vi "UDP Date Time and Match Status to RPI.vi"(6 "Address":u32, 9 "Port":u16, 10 "port":refnum<k16>) -> ()   [LabVIEW 2025]
uses:
  <vilib>/Rock Robotics/SystemInterfaces/NetworkCommunication/NetComm_MatchType.ctl
  <vilib>/Rock Robotics/WPI/DriverStation/WPI_DriverStationRobotMode2.ctl
panel:
  out "Match Type":T1
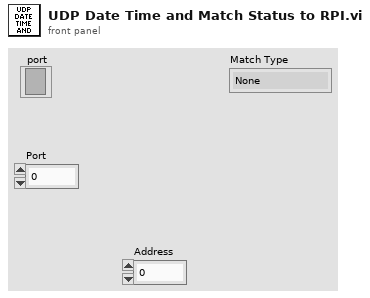
[diagram p1: front panel]
types:
  T1 = typedef "NetComm_MatchType.ctl" = enum32{"None", "Practice", "Qualification", "Elimination"}
  T2 = typedef "WPI_DriverStationRobotMode2.ctl" = enum16{"Autonomous Disabled", "Autonomous Enabled", "Teleop Disabled", "Teleop Enabled", "Disconnected", "Finish", "Test Disabled", "Test Enabled", "Emergency Stopped"}
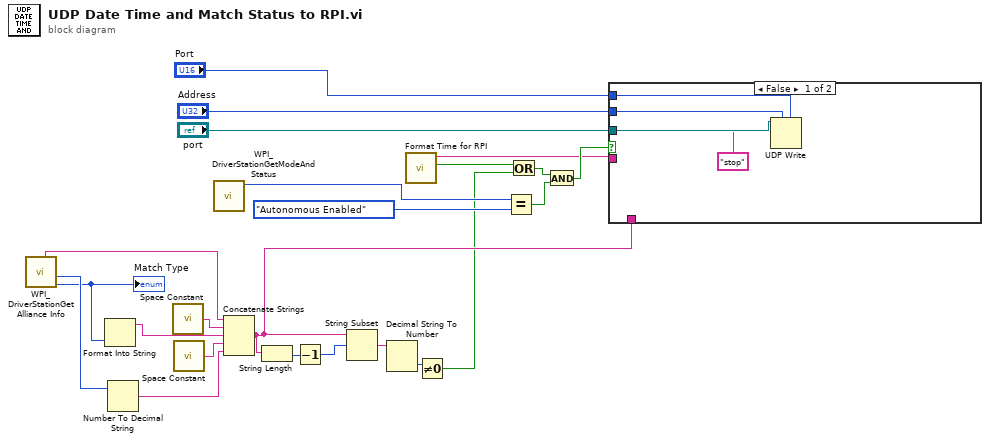
[diagram p0: block diagram]
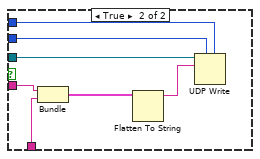
[diagram p2: hidden frame]
diagram:
  n1 = call <vilib>:"WPI_DriverStationGet Alliance Info.vi"() -> ("Match Type"=w2:T1, "Match Number"=w16:u16, "Event Name"=w13:string)  [unwired: 6 in, 3 out]
  "Match Type" <- w2
  n2 = Format Into String(w2) -> (resulting string=w1:string)  [unwired: 3 in, 1 out]
  n3 = Number To Decimal String(number=w16) -> (decimal integer string=w17:string)  [unwired: 1 in]
  n4 = call <vilib>:"Space Constant.vi"() -> ("String"=w14:string)
  n5 = call <vilib>:"Space Constant.vi"() -> ("String"=w15:string)
  n6 = call <vilib>:"WPI_DriverStationGetModeAndStatus.vi"() -> ("Robot Mode"=w20:T2)  [unwired: 10 in, 1 out]
  n7 = Concatenate Strings(w13, w14, w1, w15, w17) -> (w7:string)
  n8 = String Length(string=w7) -> (length=w8:i32)
  n9 = Decrement(x=w8) -> (x-1=w6:i32)
  n10 = String Subset(string=w7, offset (0)=w6) -> (substring=w5:string)  [unwired: 1 in]
  n11 = Decimal String To Number(string=w5) -> (number=w4:i32)  [unwired: 2 in, 1 out]
  n12 = call "Format Time for RPI.vi"() -> ("is date valid?"=w19:bool, "date/time string"=w12:string)  [unwired: 10 in]
  n13 = Not Equal To 0?(x=w4) -> (x != 0?=w3:bool)
  n14 = Equal?(x=w20, y=WPI_DriverStationRobotMode2."Autonomous Enabled") -> (x = y?=w22:bool)
  n15 = Or(x=w19, y=w3) -> (x .or. y?=w18:bool)
  n16 = And(x=w18, y=w22) -> (x .and. y?=w23:bool)
  n17 = case shown="False" w23 {
    tunnel: "Address" -> [w26 w34]
    tunnel: "Port" -> [w27 w33]
    tunnel: "port" -> [w25 w32]
    tunnel: w12 -> [_ w29]
    tunnel: w7 -> [_ w31]
    frame False {
      n18 = UDP Write(address=w26, port or service name=w27, connection ID=w25, data in="stop") -> ()  [unwired: 2 in, 2 out]
    }
    frame True {
      n19 = Bundle("date/time string"=w29, w31) -> (w30:cluster{"date/time string":string, string})  [unwired: 1 in]
      n20 = Flatten To String(anything=w30) -> (data string=w28:string)  [unwired: 3 in, 2 out]
      n21 = UDP Write(address=w34, port or service name=w33, connection ID=w32, data in=w28) -> ()  [unwired: 2 in, 2 out]
    }
  }
